vi "Update Value.vi"(6 "Time":dbl, 8 "error in (no error)":errorcluster, 11 "SystemConfigStatusIndicator in":refnum<class "SystemConfigStatusIndicator.lvclass">) -> (0 "error out":errorcluster, 1 "Update":bool, 2 "Value":variant, 3 "SystemConfigStatusIndicator out":refnum<class "SystemConfigStatusIndicator.lvclass">)   [LabVIEW 2020, in "VolatusGUIElements.lvlib" / "SystemConfigStatusIndicator.lvclass"]
uses:
  SystemConfigStatusIndicator.lvclass
  SystemConfigStatusIndicator.lvclass/SystemConfigStatusIndicator.ctl
  Volatus/System Config Status API/System Config Status API.lvclass
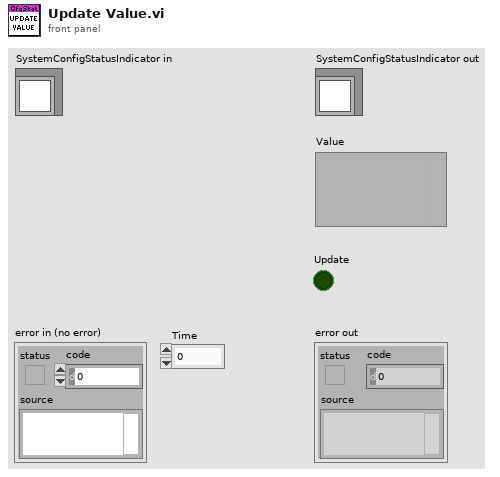
[diagram p1: front panel]
types:
  T1 = typedef "Volatus.lvlib/Config Monitor Module.lvclass/Node Config Info.ctl" = cluster{"Node":string, "Config Version":string, "Config Hash":string, "Pull":bool, "Push":bool, "Version Color":u32, "Hash Color":u32, "Node Color":u32}
  T2 = cluster{"Status Color":u32, "Status String":string, "Config GUI":bool, "Status":cluster{"Node Name":string, "Node Color":u32, "Version Color":u32, "Hash Color":u32}[]}
  T3 = cluster{"Node Name":string, "Node Color":u32, "Version Color":u32, "Hash Color":u32}
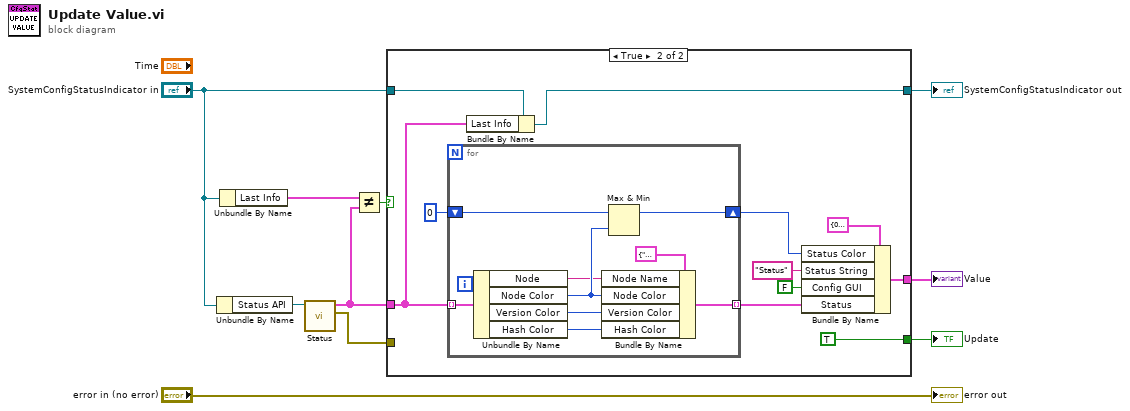
[diagram p0: block diagram]
diagram:
  n1 = Unbundle By Name("SystemConfigStatusIndicator in") -> ("Status API"=w3:refnum<class "System Config Status API.lvclass">)
  n2 = Unbundle By Name("SystemConfigStatusIndicator in") -> ("Last Info"=w8:T1[])
  n3 = call "Status.vi"("System Config Status API in"=w3) -> ("error out"=w1:errorcluster, "Config Status"=w2:T1[])  [unwired: 9 in]
  n4 = Not Equal?(x=w8, y=w2) -> (x != y?=w6:bool)
  n5 = case shown="True" w6 {
    tunnel: [_ w17] -> w9
    tunnel: w2 -> [_ w14]
    tunnel: "SystemConfigStatusIndicator in" -> [w11 w15]
    tunnel: [w11 w13] -> w5
    tunnel: [_ TRUE] -> w4
    tunnel: w1 -> [_ _]
    frame False {
    }
    frame True {
      n6 = for {
        tunnel: [w30] -> w20 mode=indexing
        tunnel: w14 -> [w29] mode=indexing
        shift-right: [w24] -> w18
        shift-left: u32 0 -> [w25]
        n7 = Unbundle By Name(w29) -> ("Node"=w23:string, "Node Color"=w26:u32, "Version Color"=w28:u32, "Hash Color"=w27:u32)
        n8 = Bundle By Name(cluster=T3 {"Node Name"="", "Node Color"=0, "Version Color"=0, "Hash Color"=0} ("Node Status"), "Node Name"=w23, "Node Color"=w26, "Version Color"=w28, "Hash Color"=w27) -> (w30:T3)
        n9 = Max & Min(x=w25, y=w26) -> (max(x,y)=w24:u32)  [unwired: 1 out]
      }
      n10 = Bundle By Name(cluster=w15, "Last Info"=w14) -> (w13:refnum<class "SystemConfigStatusIndicator.lvclass">)
      n11 = Bundle By Name(cluster=T2 {"Status Color"=0, "Status String"="", "Config GUI"=FALSE, "Status"=[]} ("System Config Status"), "Status Color"=w18, "Status String"="Status", "Config GUI"=FALSE, "Status"=w20) -> (w17:T2)
    }
  }
  "SystemConfigStatusIndicator out" <- w5
  "Value" <- w9
  "Update" <- w4
  "error out" <- "error in (no error)"
